vi "PWP Stabilization - Parse Test Type.vi"(8 "error in (no error)":errorcluster, 10 "Array":T3(array[cluster]), 11 "Cluster in":T1) -> (0 "error out":errorcluster, 1 "size(s)":i32, 3 "Cluster out":T1)   [LabVIEW 2019]
uses:
  Controls/Report - Data Structure.ctl
  <vilib>/httpClient/ClientHandle.ctl
  <vilib>/httpClient/POSTBuffer.vi
  <vilib>/httpClient/LabVIEWHTTPClient.lvlib
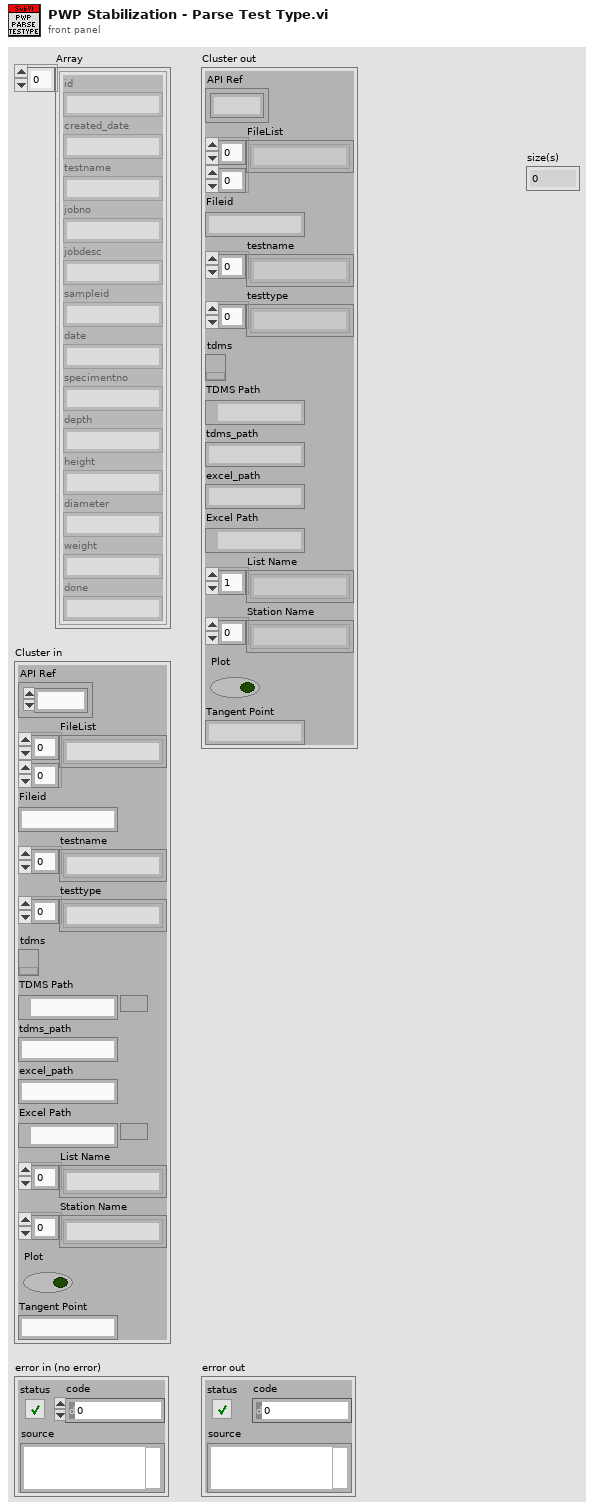
[diagram p1: front panel]
types:
  T1 = typedef "Report - Data Structure.ctl" = cluster{"API Ref":T2, "FileList":string[][], "Fileid":string, "testname":string[], "testtype":string[], "tdms":refnum<k34>, "TDMS Path":path, "tdms_path":string, "excel_path":string, "Excel Path":path, "List Name":string[], "Station Name":string[], "Plot":bool, "Tangent Point":string}
  T2 = typedef "LabVIEWHTTPClient.lvlib/ClientHandle.ctl" = refnum<k1>
  T3 = cluster{"id":string, "created_date":string, "testname":string, "jobno":string, "jobdesc":string, "sampleid":string, "date":string, "specimentno":string, "depth":string, "height":string, "diameter":string, "weight":string, "done":string}[]
  T4 = cluster{"status":string, "data":cluster{"testname":string, "testtype":string, "stage":string}[]}
  T5 = cluster{"testname":string, "testtype":string, "stage":string}[]
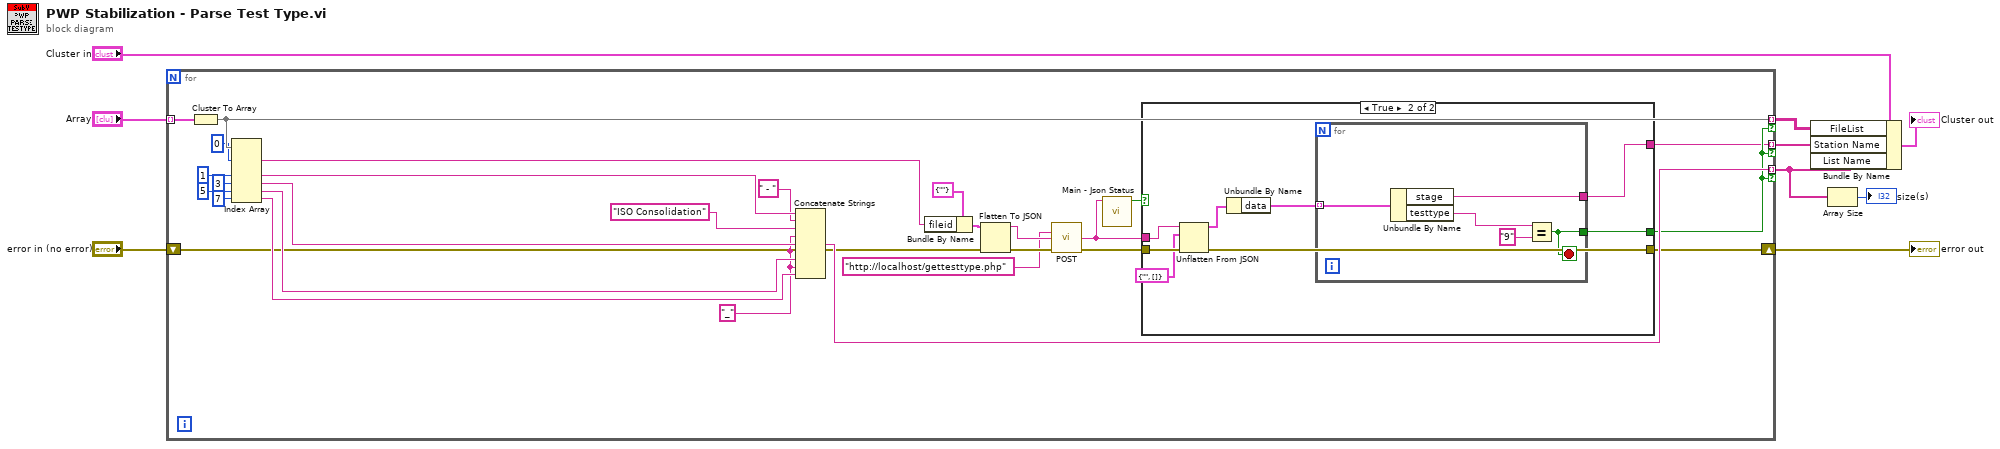
[diagram p0: block diagram]
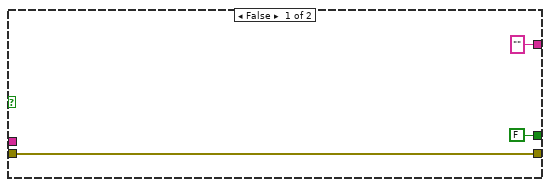
[diagram p2: hidden frame]
diagram:
  n1 = for {
    tunnel: "Array" -> [w37] mode=indexing
    tunnel: [w36] -> w4 mode=indexing if=w23
    shift-right: [w26] -> w6
    shift-left: "error in (no error)" -> [w12]
    tunnel: [w27] -> w2 mode=indexing if=w23
    tunnel: [w13] -> w7 mode=indexing if=w23
    w10 = "_" ("string")
    n2 = Cluster To Array(cluster=w37) -> (array=w36:string[])
    n3 = Index Array(array=w36, index #1=0 ("index"), index #3=1 ("index (col)"), index #4=3 ("index (col)"), index #5=5 ("index (col)"), index #6=7 ("index (col)")) -> (element #1=w24:string, element #3=w31:string, element #4=w30:string, element #5=w29:string, element #6=w28:string)  [unwired: 1 in, 1 out]
    n4 = Concatenate Strings(w31, " - " ("string"), "ISO Consolidation" ("string"), w10, w30, w10, w29, w10, w28) -> (w27:string)
    n5 = Bundle By Name(cluster=cluster{"fileid":string} {"fileid"=""}, "fileid"=w24) -> (w18:cluster{"fileid":string})
    n6 = Flatten To JSON(anything=w18, error in (no error)=w12) -> (JSON string=w20:string, 11:w19:errorcluster)  [unwired: 1 in]
    n7 = call-poly <vilib>:"POST.vi"("url"="http://localhost/gettesttype.php", "buffer"=w20, "error in (no error)"=w19) -> ("body"=w15:string, "error out"=w21:errorcluster)  [unwired: 9 in, 2 out]
    n8 = call "Main - Json Status.vi"("json"=w15) -> ("Success?"=w14:bool)  [unwired: 9 in, 1 out]
    n9 = case shown="True" w14 {
      tunnel: w21 -> [w40 w48]
      tunnel: [w40 w46] -> w26
      tunnel: [FALSE w45] -> w23
      tunnel: w15 -> [_ w44]
      tunnel: ["" ("stage") w41] -> w13
      frame False {
      }
      frame True {
        n10 = Unflatten From JSON(JSON string=w44, type and defaults=T4 {"status"="", "data"=[]}, error in (no error)=w48) -> (value=w47:T4, error out=w46:errorcluster)  [unwired: 4 in]
        n11 = Unbundle By Name(w47) -> ("data"=w42:T5)
        n12 = for {
          tunnel: [w49] -> w45
          tunnel: w42 -> [w50] mode=indexing
          tunnel: [w51] -> w41
          stop <- w49 stop-if-true
          n13 = Unbundle By Name(w50) -> ("stage"=w51:string, "testtype"=w52:string)
          n14 = Equal?(x=w52, y="9") -> (x = y?=w49:bool)
        }
      }
    }
  }
  "error out" <- w6
  n15 = Bundle By Name(cluster="Cluster in", "FileList"=w4, "Station Name"=w7, "List Name"=w2) -> (→"Cluster out":T1)
  n16 = Array Size(array=w2) -> (size(s)=→"size(s)":i32)
